vi "clone.vi"(0 "reference":refnum<class "CallNode.lvclass">, 5 "error in (no error)":errorcluster) -> (14 "reference out":refnum<class "CallNode.lvclass">, 15 "clonedCallNode":refnum<class "AbstractNode.lvclass">, 19 "error out":errorcluster)   [LabVIEW 2020, in "CallNode.lvclass"]
uses:
  <resource>/Framework/Providers/Open_GDS/UML/CallNode_class/CallNode.lvclass
  C:/Program Files (x86)/National Instruments/LabVIEW 2020/resource/Framework/Providers/Open_GDS/UML/RectangularNode_class/RectangularNode.lvclass
  C:/Program Files (x86)/National Instruments/LabVIEW 2020/resource/Framework/Providers/Open_GDS/UML/AbstractNode_class/AbstractNode.lvclass
  <resource>/Framework/Providers/Open_GDS/UML/AbstractNode_class/AbstractNode.lvclass
  <resource>/Framework/Providers/Open_GDS/UML/RectangularNode_class/RectangularNode.lvclass
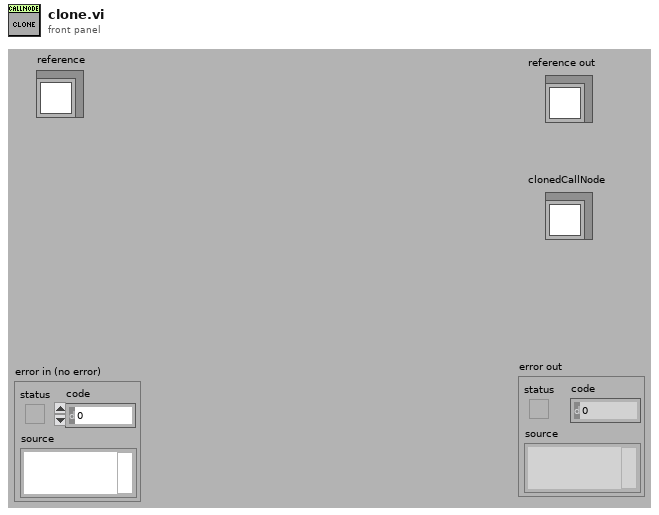
[diagram p1: front panel]
types:
  T1 = typedef "RectangularNode.lvclass/ObjectAttributes.ctl" = cluster{"bounds":T2}
  T2 = typedef "Rectangle Rectangle2D.ctl" = cluster{"x":dbl, "y":dbl, "width":dbl, "height":dbl}
  T3 = typedef "CallNode.lvclass/ObjectAttributes.ctl" = cluster{"objectCallNodeRef":refnum<class "AbstractNode.lvclass">, "signaled":bool, "openBottom":bool, "DEFAULT_WIDTH":i32, "DEFAULT_HEIGHT":i32, "CALL_YGAP":i32}
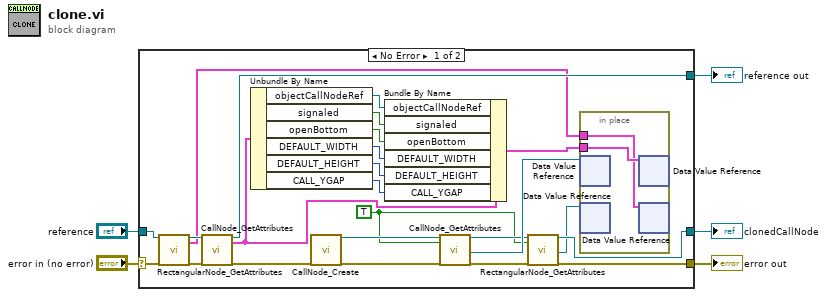
[diagram p0: block diagram]
diagram:
  n1 = case shown="No Error" "error in (no error)" {
    selector: "error in (no error)" -> [w14 w32]
    tunnel: "reference" -> [w29 w33]
    tunnel: [w9 w32] -> w3
    tunnel: [w20 w33] -> w2
    tunnel: [w10 _] -> w1
    frame No Error {
      w7 = TRUE ("OnlyGetDvrReference(False)")
      n2 = call <resource>:"RectangularNode_GetAttributes.vi"("reference in"=w29, "error in (no error)"=w14) -> ("reference out"=w15:refnum<class "CallNode.lvclass">, "Data"=w6:T1, "error out"=w13:errorcluster)  [unwired: 14 in, 1 out]
      n3 = call <resource>:"CallNode_GetAttributes.vi"("reference in"=w15, "error in (no error)"=w13) -> ("reference out"=w20:refnum<class "CallNode.lvclass">, "Data"=w18:T3, "error out"=w21:errorcluster)  [unwired: 1 in, 14 out]
      n4 = Unbundle By Name(w18) -> ("objectCallNodeRef"=w28:refnum<class "AbstractNode.lvclass">, "signaled"=w27:bool, "openBottom"=w26:bool, "DEFAULT_WIDTH"=w25:i32, "DEFAULT_HEIGHT"=w24:i32, "CALL_YGAP"=w23:i32)
      n5 = call <resource>:"CallNode_Create.vi"("error in (no error)"=w21) -> ("reference out"=w19:refnum<class "CallNode.lvclass">, "error out"=w22:errorcluster)  [unwired: 17 in]
      n6 = Bundle By Name(cluster=w18, "objectCallNodeRef"=w28, "signaled"=w27, "openBottom"=w26, "DEFAULT_WIDTH"=w25, "DEFAULT_HEIGHT"=w24, "CALL_YGAP"=w23) -> (w16:T3)
      n7 = call <resource>:"CallNode_GetAttributes.vi"("reference in"=w19, "OnlyGetDvrReference(False)"=w7, "error in (no error)"=w22) -> ("reference out"=w12:refnum<class "CallNode.lvclass">, "DataRef"=w17:refnum<data-value>, "error out"=w11:errorcluster)  [unwired: 13 in, 1 out]
      n8 = call <resource>:"RectangularNode_GetAttributes.vi"("reference in"=w12, "OnlyGetDvrReference(False)"=w7, "error in (no error)"=w11) -> ("reference out"=w10:refnum<class "CallNode.lvclass">, "DataRef"=w8:refnum<data-value>, "error out"=w9:errorcluster)  [unwired: 13 in, 1 out]
      n9 = in-place {
        in-place-border: w16 -> [w31]
        in-place-border: w6 -> [w30]
        n10 = in-place-dvr #1(w17) -> ()  [unwired: 2 out]
        n11 = in-place-dvr #2(w8) -> ()  [unwired: 2 out]
        n12 = in-place-dvr #1(w31) -> ()  [unwired: 2 out]
        n13 = in-place-dvr #2(w30) -> ()  [unwired: 2 out]
      }
    }
    frame Error {
    }
  }
  "reference out" <- w2
  "error out" <- w3
  "clonedCallNode" <- w1
